vi "Message sauvegarde perdu.vi"() -> ()   [LabVIEW 2022 SP3]
uses:
  Variables globales/Variable glob generale.vi
panel:
  out "Chemin":path
  in  "Bouton OK":bool
  # "la communication avec\nle poste SAUVEGARDE :"
  # "a été perdue\nvérifier la liaison réseau"
  # "Ce logiciel et les informations qu'il contient, sont la propriété de l’IAS \net ne peuvent être diffusés sans l’autorisation de la Station d’étalonnage"
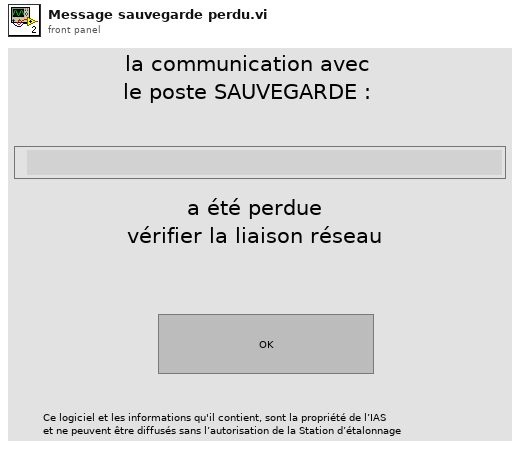
[diagram p1: front panel]
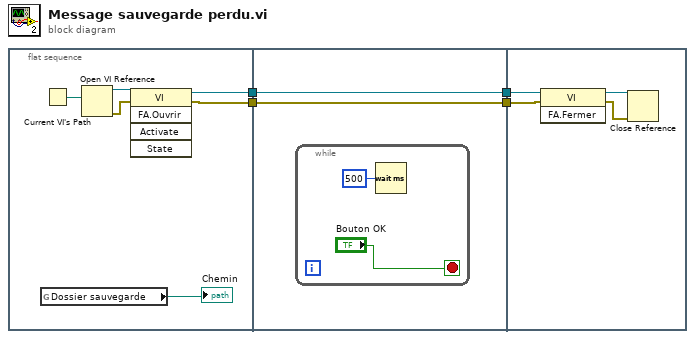
[diagram p0: block diagram]
diagram:
  n1 = flat-sequence {
    tunnel: [w7] -> w4
    tunnel: [w5] -> w1
    tunnel: w4 -> [w12]
    tunnel: [w12] -> w3
    tunnel: [w11] -> w2
    tunnel: w1 -> [w11]
    tunnel: w3 -> [w18]
    tunnel: w2 -> [w15]
    frame #0 {
      n2 = global read "Variable glob generale.vi" "Dossier sauvegarde"() -> (→"Chemin":path)
      n3 = Current VI's Path() -> (path=w8:path)
      n4 = Open VI Reference(vi path=w8) -> (vi reference=w9:refnum<vi>, error out=w10:errorcluster)  [unwired: 5 in]
      n5 = invoke class="VI" method="FA.Ouvrir"(reference=w9, error in=w10) -> (reference out=w7:refnum<vi>, error out=w5:errorcluster)  [unwired: 3 in, 3 out]
    }
    frame #1 {
      n6 = while {
        stop <- "Bouton OK" stop-if-true
        n7 = Wait (ms)(milliseconds to wait=u32 500 ("attente (ms)")) -> ()  [unwired: 1 out]
      }
    }
    frame #2 {
      n8 = invoke class="VI" method="FA.Fermer"(reference=w18, error in=w15) -> (reference out=w16:refnum<vi>, error out=w17:errorcluster)  [unwired: 1 in, 1 out]
      n9 = Close Reference(reference=w16, error in (no error)=w17) -> ()  [unwired: 1 out]
    }
  }
